vi "Calculate Nominal Resistance.vi"(8 "error in (no error)":errorcluster, 10 "Number of Bands":T6=4 min=3 max=6 step=1, 11 "Selectors":T1={"1Dig"=enum."Black - 0", "2Dig"=enum."Black - 0", "3Dig"=enum."Black - 0", "Mul"=enum."Silver - x 0.01", "Tol"=enum."Gold - 5%", "TC"=enum."Grey - 1 ppm/K"}) -> (0 "error out":errorcluster, 3 "Nominal Value":dbl format="%#_2p")   [LabVIEW 2018, in "Resistance Value.lvlib"]
doc: "Calculates the nominal resistance value from the resistor band selections and number of bands.\n\nThe VI receives the <b>Selectors</b> cluster and the <b>Number of Bands</b>. It uses <b>Build Resistor Ciphers.vi</b> to construct the integer value represented by the significant digits, then uses <b>Determine Multiplier Value.vi</b> to obtain the numerical multiplier corresponding to the selected multiplier color.\n\nThe nominal resistance is calculated by multiplying the significant value by the numerical multiplier.\n\nThe resulting value is returned through <b>Nominal Value</b>. The VI propagates errors through its <b>error in</b> and <b>error out</b> terminals."
uses:
  Resistance Value.lvlib
  Number of Bands--numeric.ctl
  Resistor Controls/Selectors--cluster.ctl
  Resistor Controls/Digit--enum.ctl
  Resistor Controls/Multiplier--enum.ctl
  Resistor Controls/Tolerance--enum.ctl
  Resistor Controls/Temp Coefficient--enum.ctl
  Resistor Controls/Resistance Controls.lvlib
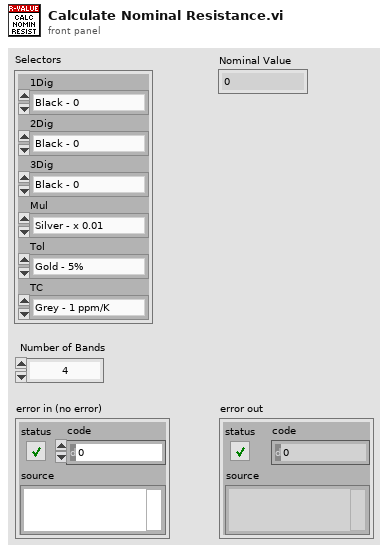
[diagram p1: front panel]
types:
  T1 = typedef "Resistance Controls.lvlib/Selectors--cluster.ctl" = cluster{"1Dig":T2, "2Dig":T2, "3Dig":T2, "Mul":T3, "Tol":T4, "TC":T5}
  T2 = typedef "Resistance Controls.lvlib/Digit--enum.ctl" = enum16{"Black - 0", "Brown - 1", "Red - 2", "Orange - 3", "Yellow - 4", "Green - 5", "Blue - 6", "Violet - 7", "Grey - 8", "White - 9"}
  T3 = typedef "Resistance Controls.lvlib/Multiplier--enum.ctl" = enum16{"Silver - x 0.01", "Gold - x 0.1 ", "Black - x 1", "Brown - x 10", "Red - x 100", "Orange - x 1k", "Yellow - x 10k", "Green - 100k", "Blue - x 1M", "Violet - x10 M", "Grey - x 100M", "White - x 1G"}
  T4 = typedef "Resistance Controls.lvlib/Tolerance--enum.ctl" = enum16{"Gray - 0.05%", "Violet - 0.1%", "Blue - 0.25%", "Green - 0.5%", "Brown - 1%", "Red - 2%", "Gold - 5%", "Silver - 10%", "None - 20%"}
  T5 = typedef "Resistance Controls.lvlib/Temp Coefficient--enum.ctl" = enum16{"Grey - 1 ppm/K", "Violet - 5 ppm/K", "Blue - 10 ppm/K", "Green - 20 ppm/K", "Yellow - 25 ppm/K", "Orange - 15 ppm/K", "Red - 50 ppm/K", "Brown - 100 ppm/K", "Black - 250 ppm/K"}
  T6 = typedef "Number of Bands--numeric.ctl" = u8
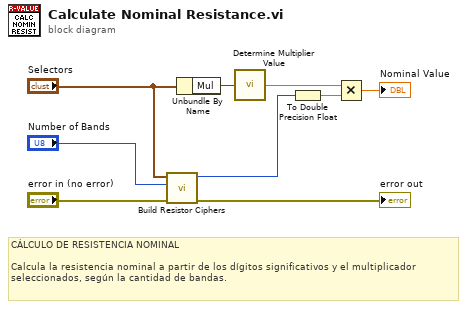
[diagram p0: block diagram]
diagram:
  # "CÁLCULO DE RESISTENCIA NOMINAL\n\nCalcula la resistencia nominal a partir de los dígitos significativos y el multiplicador seleccionados, según la cantidad de bandas."
  n1 = call "Build Resistor Ciphers.vi"("error in (no error)"="error in (no error)", "Number of Bands"="Number of Bands", "Selectors"="Selectors") -> ("error out"=→"error out":errorcluster, "Nominal Value"=w6:i32)  [unwired: 6 in, 1 out]
  n2 = Unbundle By Name("Selectors") -> ("Mul"=w2:T3)
  n3 = call "Determine Multiplier Value.vi"("mult color"=w2) -> ("multiplier"=w7:dbl)  [unwired: 6 in]
  n4 = To Double Precision Float(number=w6) -> (double precision float=w8:dbl)
  n5 = Multiply(x=w7, y=w8) -> (x*y=→"Nominal Value":dbl)
